vi "LABVIEW MODBUS.vi"() -> ()   [LabVIEW 2021]
uses:
  <vilib>/Modbus/master/Create Master Instance (Serial).vi
  <vilib>/Modbus/master/Modbus Master.lvclass
panel:
  out "Meter":dbl(knob) scale=0.0..100.0
  out "Thermometer":dbl(slide) scale=0.0..100.0
  in  "stop":bool
  out "register values":u16[](array[numeric])
  in  "number of input registers":u16
  in  "starting address":u16
  in  "VISA resource name":refnum<visa-resource-name>
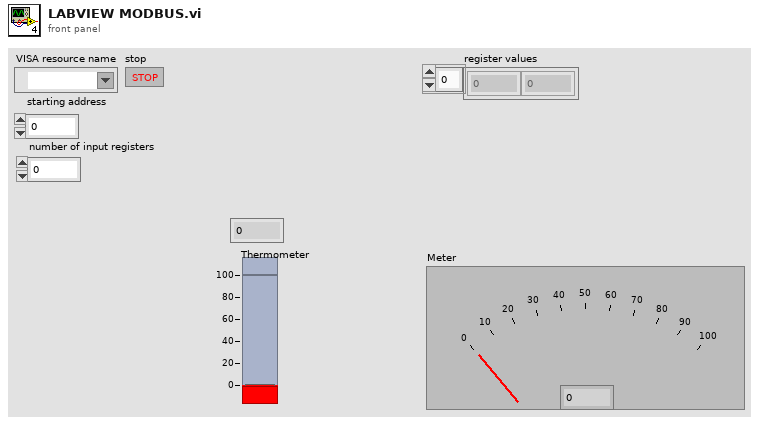
[diagram p1: front panel]
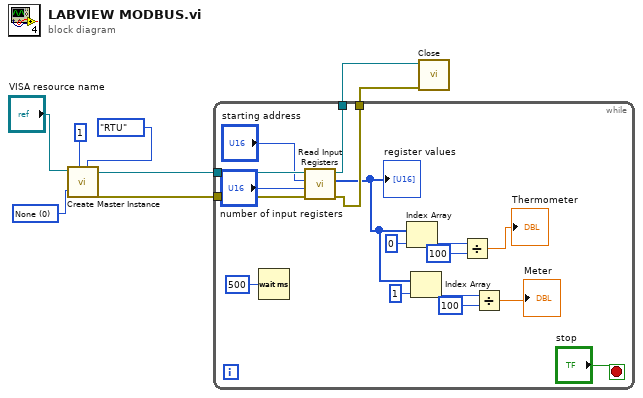
[diagram p0: block diagram]
diagram:
  w6 = u16 0 items=["None", "Odd", "Even"] ("parity (Even)")
  n1 = call-poly <vilib>:"Create Master Instance.vi"("serial type"=enum16{"RTU", "ASCII"}."RTU", "parity (Even)"=w6, "unit ID"=u8 1, "VISA resource name"="VISA resource name") -> ("error out"=w4:errorcluster, "serial master instance"=w5:refnum<class "Modbus Master.lvclass">)  [unwired: 6 in]
  n2 = while {
    tunnel: w5 -> [w25]
    tunnel: w4 -> [w24]
    tunnel: [w20] -> w3
    tunnel: [w19] -> w2
    stop <- "stop" stop-if-true
    n3 = Wait (ms)(milliseconds to wait=u32 500) -> ()  [unwired: 1 out]
    n4 = call-dynamic "Read Input Registers.vi"("error in (no error)"=w24, "number of input registers"="number of input registers", "starting address"="starting address", "Modbus master in"=w25) -> ("error out"=w20:errorcluster, "register values"=w15:u16[], "Modbus master out"=w19:refnum<class "Modbus Master.lvclass">)  [unwired: 5 in]
    "register values" <- w15
    n5 = Index Array(array=w15, index=0) -> (element=w14:u16)
    n6 = Index Array(array=w15, index=1) -> (element=w10:u16)
    n7 = Divide(x=w14, y=u16 100) -> (x/y=→"Thermometer":dbl)
    n8 = Divide(x=w10, y=u16 100) -> (x/y=→"Meter":dbl)
  }
  n9 = call-dynamic "Close.vi"("error in (no error)"=w3, "Modbus master in"=w2) -> ()  [unwired: 9 in, 1 out]
